vi "Post-Build Custom Action.vi"(10 "Variant":variant) -> (0 "error out":errorcluster)   [LabVIEW 2020]
doc: "VIPM Post-Build action. Re-saves any VI in the built package that is not saved in LabVIEW 2020 (see Save Package For Previous.vi)."
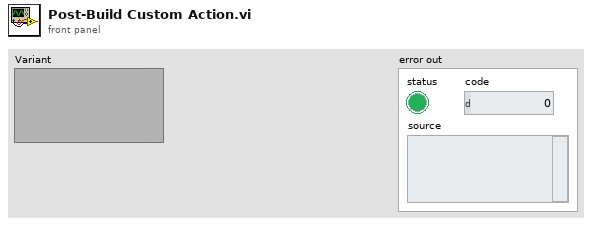
[diagram p1: front panel]
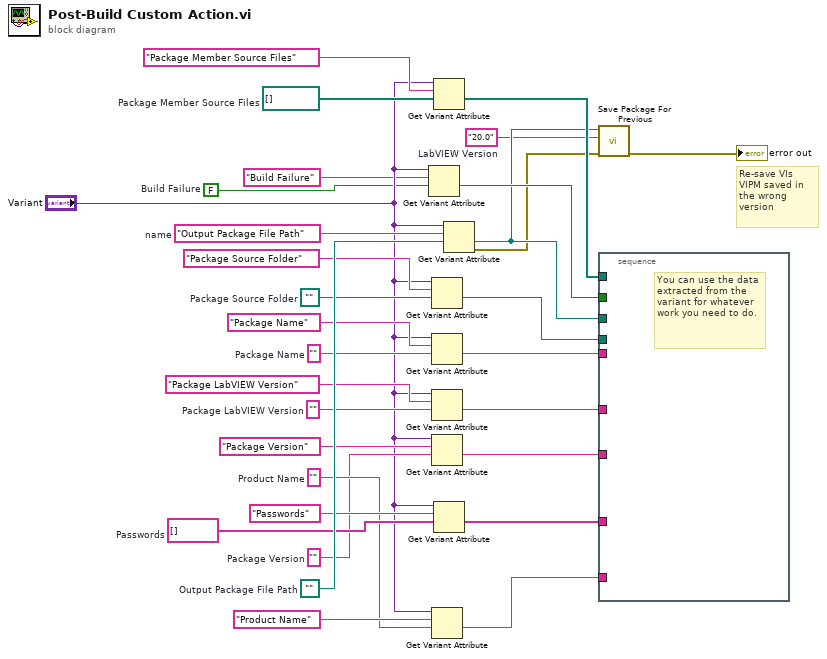
[diagram p0: block diagram]
diagram:
  w3 = "20.0"  # LabVIEW Version
  w13 = FALSE  # Build Failure
  w16 = path ""  # Package Source Folder
  w18 = ""  # Package Name
  w20 = ""  # Package LabVIEW Version
  w22 = ""  # Package Version
  w24 = ""  # Product Name
  w26 = string[] []  # Passwords
  w28 = path[] []  # Package Member Source Files
  w30 = path ""  # Output Package File Path
  w31 = "Output Package File Path"  # name
  # "Re-save VIs VIPM saved in the wrong version"
  n1 = Get Variant Attribute(Variant="Variant", name="Build Failure", default value (empty Variant)=w13) -> (value=w5:bool)  [unwired: 1 in, 3 out]
  n2 = Get Variant Attribute(Variant="Variant", name="Package Source Folder", default value (empty Variant)=w16) -> (value=w7:path)  [unwired: 1 in, 3 out]
  n3 = Get Variant Attribute(Variant="Variant", name="Package Name", default value (empty Variant)=w18) -> (value=w6:string)  [unwired: 1 in, 3 out]
  n4 = Get Variant Attribute(Variant="Variant", name="Package LabVIEW Version", default value (empty Variant)=w20) -> (value=w8:string)  [unwired: 1 in, 3 out]
  n5 = Get Variant Attribute(Variant="Variant", name="Package Version", default value (empty Variant)=w22) -> (value=w9:string)  [unwired: 1 in, 3 out]
  n6 = Get Variant Attribute(Variant="Variant", name="Product Name", default value (empty Variant)=w24) -> (value=w10:string)  [unwired: 1 in, 3 out]
  n7 = Get Variant Attribute(Variant="Variant", name="Package Member Source Files", default value (empty Variant)=w28) -> (value=w12:path[])  [unwired: 1 in, 3 out]
  n8 = Get Variant Attribute(Variant="Variant", name="Passwords", default value (empty Variant)=w26) -> (value=w11:string[])  [unwired: 1 in, 3 out]
  n9 = Get Variant Attribute(Variant="Variant", name=w31, default value (empty Variant)=w30) -> (value=w4:path, error out=w2:errorcluster)  [unwired: 1 in, 2 out]
  n10 = call "Save Package For Previous.vi"("error in (no error)"=w2, "LabVIEW Version"=w3, "Package File"=w4) -> ("error out"=→"error out":errorcluster)  [unwired: 7 in, 1 out]
  n11 = stacked-sequence {
    tunnel: w4 -> [_]
    tunnel: w12 -> [_]
    tunnel: w11 -> [_]
    tunnel: w10 -> [_]
    tunnel: w9 -> [_]
    tunnel: w8 -> [_]
    tunnel: w7 -> [_]
    tunnel: w6 -> [_]
    tunnel: w5 -> [_]
    frame #0 {
      # "You can use the data extracted from the variant for whatever work you need to do."
    }
  }
